vi "find_midle_lane_v3.vi"(8 "max_cluster_size":dbl=150.0 format="%#_13g", 9 "euclid":dbl=110.0, 10 "LiDAR_Y":i32[](array[numeric]), 11 "LiDAR_X":i32[](array[numeric])) -> (0 "크기":i32, 1 "lidar_x":dbl=-0.4638235294117647, 2 "ladpoint":cluster{dbl[], dbl[]}(graph)={[-463.8235294117647], [1690.0]}, 3 "filtered_data":cluster{dbl[], dbl[]}(graph)={[0.0, 0.0, 0.0, 0.0, 0.0, 0.0, 0.0, 0.0, 0.0, 0.0, 0.0, 0.0, 0.0, 0.0, 0.0, 0.0, 0.0, 200.0, 205.0, 210.0, 0.0, 0.0, 0.0, 0.0, 0.0, 0.0, 0.0, 0.0, 0.0, 0.0, 0.0, 0.0, 0.0, 0.0], [0.0, 0.0, 0.0, 0.0, 0.0, 0.0, 0.0, 0.0, 0.0, 0.0, 0.0, 0.0, 0.0, 0.0, 0.0, 0.0, 0.0, 500.0, 500.0, 500.0, 0.0, 0.0, 0.0, 0.0, 0.0, 0.0, 0.0, 0.0, 0.0, 0.0, 0.0, 0.0, 0.0, 0.0]}, 4 "right_point":dbl=-0.4638235294117647, 6 "left_point":dbl=-0.4638235294117647)   [LabVIEW 2024]
uses:
  <vilib>/Analysis/baseanly.llb/Mean (DBL).vi
  <vilib>/Analysis/NI_AALBase.lvlib
panel:
  out "raw_data":cluster{dbl[], dbl[]}(graph)
  out "배열":bool[](array[boolean])
  out "clustered_data1":cluster{dbl[], dbl[]}[](graph)=[{[0.0, 0.0, 0.0, 0.0, 0.0, 0.0, 0.0, 0.0, 0.0, 0.0, 0.0, 0.0, 0.0, 0.0, 0.0, 0.0, 0.0], [0.0, 0.0, 0.0, 0.0, 0.0, 0.0, 0.0, 0.0, 0.0, 0.0, 0.0, 0.0, 0.0, 0.0, 0.0, 0.0, 0.0]}, {[-600.0, -605.0, -400.0, -405.0, -200.0, -205.0, 0.0, 0.0, 0.0, 0.0, 0.0, 0.0, 0.0, 0.0, 0.0, 0.0, 0.0], [500.0, 500.0, 500.0, 500.0, 500.0, 500.0, 0.0, 0.0, 0.0, 0.0, 0.0, 0.0, 0.0, 0.0, 0.0, 0.0, 0.0]}, {[200.0, 205.0, 210.0, 0.0, 0.0, 0.0, 0.0, 0.0, 0.0, 0.0, 0.0, 0.0, 0.0, 0.0, 0.0, 0.0, 0.0], [500.0, 500.0, 500.0, 0.0, 0.0, 0.0, 0.0, 0.0, 0.0, 0.0, 0.0, 0.0, 0.0, 0.0, 0.0, 0.0, 0.0]}, {[500.0, 500.0, 500.0, 500.0, 500.0, 500.0, 500.0, 500.0, 500.0, 500.0, 500.0, 500.0, 500.0, 500.0, 500.0, 500.0, 500.0], [500.0, 700.0, 710.0, 720.0, 730.0, 740.0, 750.0, 760.0, 770.0, 780.0, 790.0, 800.0, 810.0, 820.0, 830.0, 840.0, 850.0]}, {[-250.0, -280.0, -290.0, -310.0, -330.0, -340.0, -360.0, -390.0, -410.0, -430.0, -440.0, 0.0, 0.0, 0.0, 0.0, 0.0, 0.0], [1100.0, 1100.0, 1100.0, 1100.0, 1100.0, 1100.0, 1100.0, 1100.0, 1100.0, 1100.0, 1100.0, 0.0, 0.0, 0.0, 0.0, 0.0, 0.0]}]
  out "clustered_data2":cluster{dbl[], dbl[]}(graph)={[0.0, 0.0, 0.0, 0.0, 0.0, 0.0, 0.0, 0.0, 0.0, 0.0, 0.0, 0.0, 0.0, 0.0, 0.0, 0.0, 0.0, 200.0, 205.0, 210.0, 0.0, 0.0, 0.0, 0.0, 0.0, 0.0, 0.0, 0.0, 0.0, 0.0, 0.0, 0.0, 0.0, 0.0], [0.0, 0.0, 0.0, 0.0, 0.0, 0.0, 0.0, 0.0, 0.0, 0.0, 0.0, 0.0, 0.0, 0.0, 0.0, 0.0, 0.0, 500.0, 500.0, 500.0, 0.0, 0.0, 0.0, 0.0, 0.0, 0.0, 0.0, 0.0, 0.0, 0.0, 0.0, 0.0, 0.0, 0.0]}
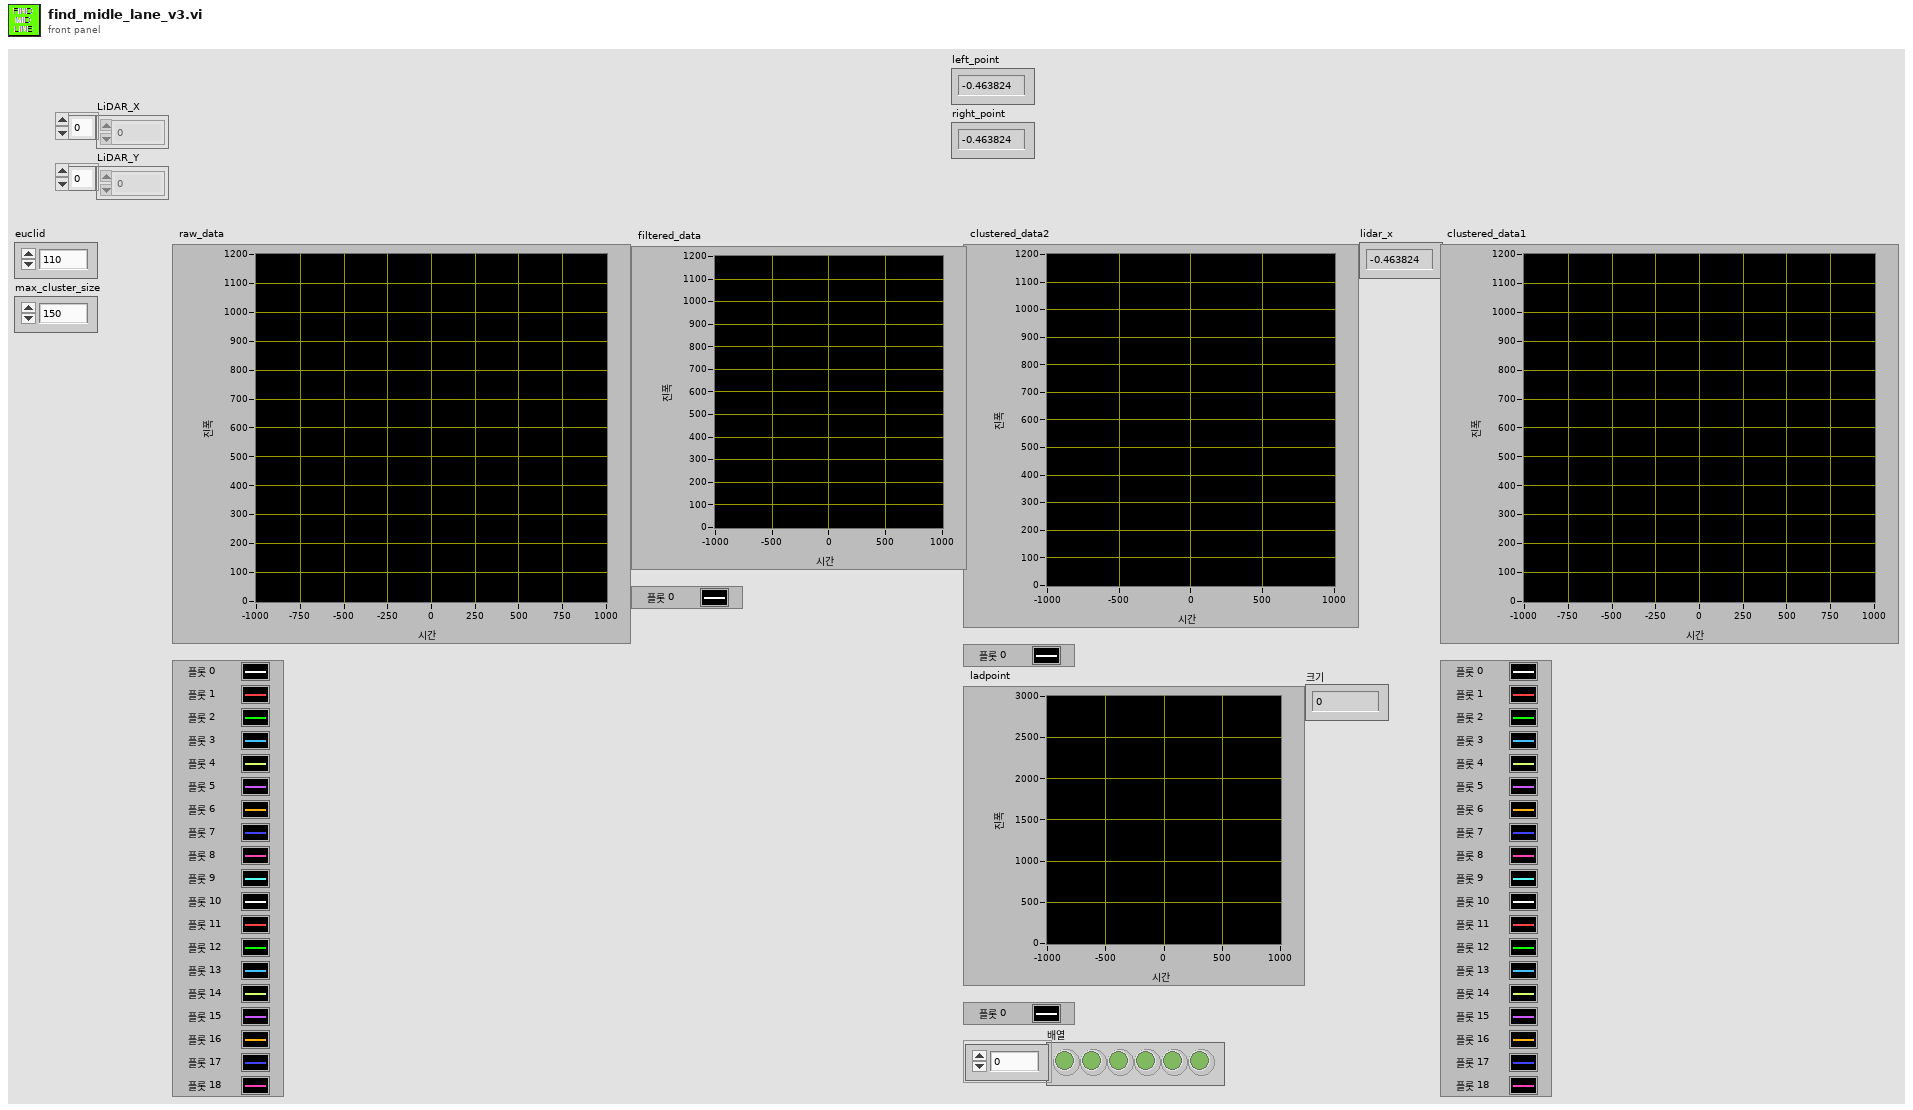
[diagram p1: front panel]
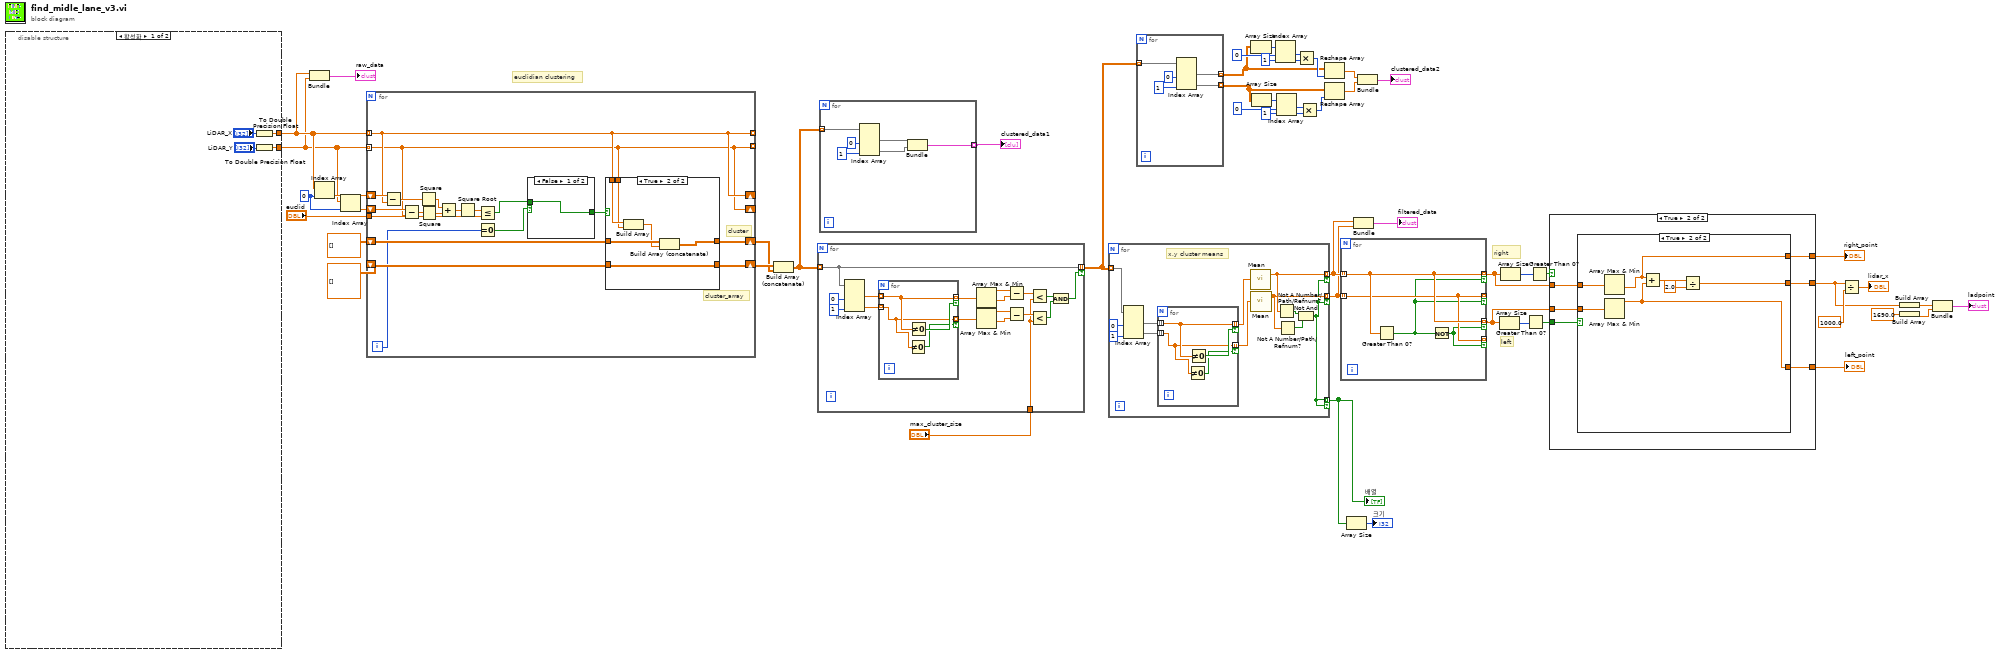
[diagram p0: block diagram]
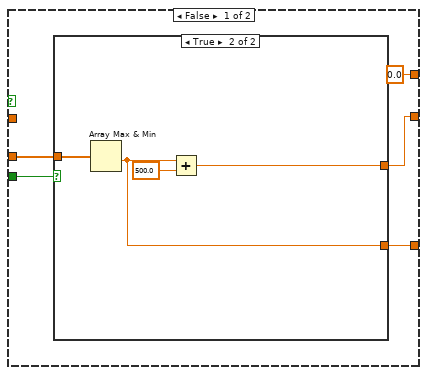
[diagram p2: hidden frame]
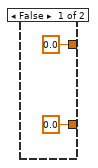
[diagram p3: hidden frame]
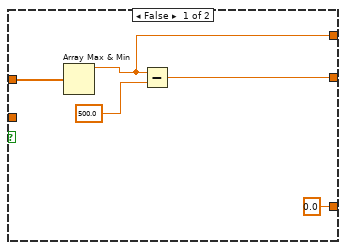
[diagram p4: hidden frame]
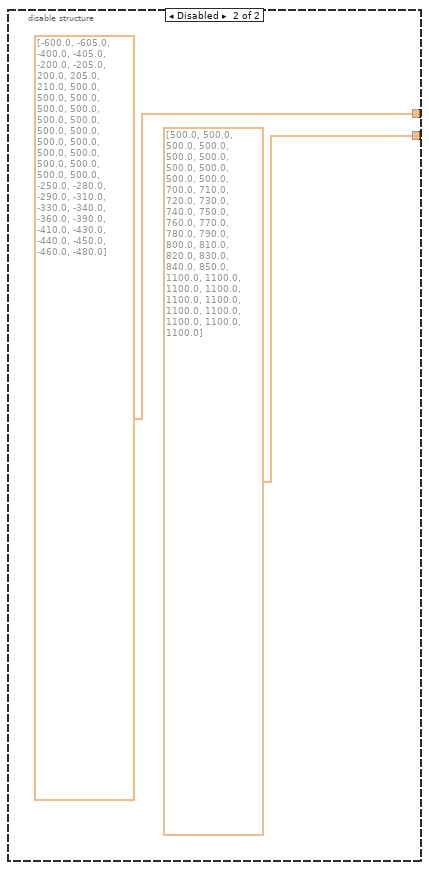
[diagram p5: hidden frame]
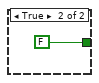
[diagram p6: hidden frame]
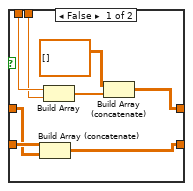
[diagram p7: hidden frame]
diagram:
  w47 = 0 ("인덱스")
  # "left"
  # "right"
  # "euclidian clustering"
  n1 = disable-structure shown="활성화" {
    disable-tunnel: [w54 dbl[] [500.0, 500.0, 500.0, 500.0, 500.0, 500.0, 500.0, 500.0, 500.0, 500.0, 700.0, 710.0, 720.0, 730.0, 740.0, 750.0, 760.0, 770.0, 780.0, 790.0, 800.0, 810.0, 820.0, 830.0, 840.0, 850.0, 1100.0, 1100.0, 1100.0, 1100.0, 1100.0, 1100.0, 1100.0, 1100.0, 1100.0, 1100.0, 1100.0]] -> w8
    disable-tunnel: [w53 dbl[] [-600.0, -605.0, -400.0, -405.0, -200.0, -205.0, 200.0, 205.0, 210.0, 500.0, 500.0, 500.0, 500.0, 500.0, 500.0, 500.0, 500.0, 500.0, 500.0, 500.0, 500.0, 500.0, 500.0, 500.0, 500.0, 500.0, -250.0, -280.0, -290.0, -310.0, -330.0, -340.0, -360.0, -390.0, -410.0, -430.0, -440.0, -450.0, -460.0, -480.0]] -> w9
    frame Enabled {
      n2 = To Double Precision Float(number="LiDAR_X") -> (double precision float=w53:dbl[])
      n3 = To Double Precision Float(number="LiDAR_Y") -> (double precision float=w54:dbl[])
    }
    frame Disabled {
    }
  }
  n4 = Bundle(w9, w8) -> (→"raw_data":cluster{dbl[], dbl[]})  [unwired: 1 in]
  n5 = Index Array(array=w9, index=w47) -> (element=w49:dbl)
  n6 = Index Array(array=w8, index=w47) -> (element=w48:dbl)
  n7 = for {
    tunnel: w9 -> [w66] mode=indexing
    tunnel: w8 -> [w65] mode=indexing
    tunnel: [w66] -> _ mode=indexing
    tunnel: [w65] -> _ mode=indexing
    shift-right: [w66] -> _
    shift-left: w49 -> [w77]
    shift-right: [w65] -> _
    shift-left: w48 -> [w76]
    tunnel: "euclid" -> [w69]
    shift-right: [w68] -> w30
    shift-left: dbl[][] [] -> [w67]
    shift-right: [w59] -> w31
    shift-left: dbl[][][] [] -> [w64]
    i -> [w63]
    # "cluster_array"
    # "cluster"
    n8 = Subtract(x=w77, y=w66) -> (x-y=w75:dbl)
    n9 = Subtract(x=w76, y=w65) -> (x-y=w74:dbl)
    n10 = Square(x=w75) -> (x^2=w73:dbl)
    n11 = Square(x=w74) -> (x^2=w72:dbl)
    n12 = Add(x=w73, y=w72) -> (x+y=w71:dbl)
    n13 = Square Root(x=w71) -> (sqrt(x)=w70:dbl)
    n14 = Equal To 0?(x=w63) -> (x = 0?=w62:bool)
    n15 = Less Or Equal?(x=w70, y=w69) -> (x <= y?=w60:bool)
    n16 = case shown="False" w62 {
      tunnel: [w78 FALSE] -> w61
      tunnel: w60 -> [w78 _]
      frame False {
      }
      frame True {
      }
    }
    n17 = case shown="True" w61 {
      tunnel: [w83 w93] -> w68
      tunnel: w67 -> [w81 w92]
      tunnel: [w80 w88] -> w59
      tunnel: w66 -> [w86 w91]
      tunnel: w65 -> [w85 w90]
      tunnel: w64 -> [w82 w88]
      frame False {
        n18 = Build Array (concatenate)(w82, w81) -> (w80:dbl[][][])
        n19 = Build Array(w86, w85) -> (w84:dbl[])
        n20 = Build Array (concatenate)(dbl[][] [], w84) -> (w83:dbl[][])
      }
      frame True {
        n21 = Build Array(w91, w90) -> (w89:dbl[])
        n22 = Build Array (concatenate)(w92, w89) -> (w93:dbl[][])
      }
    }
  }
  n23 = Build Array (concatenate)(w31, w30) -> (w16:dbl[][][])
  n24 = for {
    tunnel: w16 -> [w106] mode=indexing
    tunnel: [w106] -> w6 mode=indexing if=w101
    tunnel: "max_cluster_size" -> [w94]
    n25 = Index Array(array=w106, index (col) #1=0 ("비활성화된 인덱스 (열)"), index (col) #2=1 ("인덱스 (열)")) -> (element #1=w98:dbl[], element #2=w97:dbl[])  [unwired: 2 in]
    n26 = for {
      tunnel: w98 -> [w114] mode=indexing
      tunnel: w97 -> [w112] mode=indexing
      tunnel: [w114] -> w96 mode=indexing if=w113
      tunnel: [w112] -> w95 mode=indexing if=w111
      n27 = Not Equal To 0?(x=w112) -> (x != 0?=w111:bool)
      n28 = Not Equal To 0?(x=w114) -> (x != 0?=w113:bool)
    }
    n29 = Array Max & Min(array=w95) -> (max value=w103:dbl, min value=w102:dbl)  [unwired: 2 out]
    n30 = Array Max & Min(array=w96) -> (max value=w105:dbl, min value=w104:dbl)  [unwired: 2 out]
    n31 = Subtract(x=w105, y=w104) -> (x-y=w100:dbl)
    n32 = Subtract(x=w103, y=w102) -> (x-y=w99:dbl)
    n33 = Less?(x=w100, y=w94) -> (x < y?=w108:bool)
    n34 = Less?(x=w99, y=w94) -> (x < y?=w107:bool)
    n35 = And(x=w108, y=w107) -> (x .and. y?=w101:bool)
  }
  n36 = for {
    tunnel: w16 -> [w120] mode=indexing
    tunnel: [w115] -> w17 mode=indexing
    n37 = Index Array(array=w120, index (col) #1=0 ("인덱스"), index (col) #2=1 ("인덱스")) -> (element #1=w117:dbl[], element #2=w116:dbl[])  [unwired: 2 in]
    n38 = Bundle(w117, w116) -> (w115:cluster{dbl[], dbl[]})  [unwired: 1 in]
  }
  "clustered_data1" <- w17
  n39 = for {
    tunnel: w6 -> [w128] mode=indexing
    tunnel: [w125] -> w14 mode=indexing if=w121
    tunnel: [w124] -> w13 mode=indexing if=w121
    tunnel: [w121] -> w11 mode=indexing if=w121
    # "x,y cluster means"
    n40 = Index Array(array=w128, index (col) #1=0 ("비활성화된 인덱스 (열)"), index (col) #2=1 ("인덱스 (열)")) -> (element #1=w131:dbl[], element #2=w132:dbl[])  [unwired: 2 in]
    n41 = for {
      tunnel: w131 -> [w136] mode=indexing
      tunnel: w132 -> [w134] mode=indexing
      tunnel: [w136] -> w127 mode=indexing if=w135
      tunnel: [w134] -> w126 mode=indexing if=w133
      n42 = Not Equal To 0?(x=w134) -> (x != 0?=w133:bool)
      n43 = Not Equal To 0?(x=w136) -> (x != 0?=w135:bool)
    }
    n44 = call-poly <vilib>:"Mean.vi"("X"=w127) -> ("mean"=w125:dbl)  [unwired: 1 out]
    n45 = call-poly <vilib>:"Mean.vi"("X"=w126) -> ("mean"=w124:dbl)  [unwired: 1 out]
    n46 = Not A Number/Path/Refnum?(number/path/refnum=w125) -> (NaN/Path/Refnum?=w123:bool)
    n47 = Not A Number/Path/Refnum?(number/path/refnum=w124) -> (NaN/Path/Refnum?=w122:bool)
    n48 = Not And(1:w122, 2:w123) -> (0:w121:bool)
  }
  "배열" <- w11
  n49 = for {
    tunnel: w6 -> [w141] mode=indexing
    tunnel: [w138] -> w19 mode=indexing
    tunnel: [w137] -> w18 mode=indexing
    n50 = Index Array(array=w141, index (col) #1=0 ("인덱스"), index (col) #2=1 ("인덱스")) -> (element #1=w138:dbl[], element #2=w137:dbl[])  [unwired: 2 in]
  }
  n51 = Array Size(array=w19) -> (size(s)=w44:i32[])
  n52 = Array Size(array=w18) -> (size(s)=w39:i32[])
  n53 = Index Array(array=w44, index #1=0 ("인덱스"), index #2=1 ("인덱스")) -> (element #1=w34:i32, element #2=w35:i32)
  n54 = Index Array(array=w39, index #1=0 ("인덱스"), index #2=1 ("인덱스")) -> (element #1=w38:i32, element #2=w37:i32)
  n55 = Multiply(x=w34, y=w35) -> (x*y=w33:i32)
  n56 = Multiply(x=w38, y=w37) -> (x*y=w36:i32)
  n57 = Reshape Array(w19, w33) -> (w46:dbl[])
  n58 = Reshape Array(w18, w36) -> (w45:dbl[])
  n59 = for {
    tunnel: w14 -> [w145] mode=indexing
    tunnel: w13 -> [w144] mode=indexing
    tunnel: [w145] -> w5 mode=indexing if=w143
    tunnel: [w144] -> _ mode=indexing if=w143
    tunnel: [w145] -> w4 mode=indexing if=w142
    tunnel: [w144] -> _ mode=indexing if=w142
    n60 = Greater Than 0?(x=w145) -> (x > 0?=w143:bool)
    n61 = Not(x=w143) -> (.not. x?=w142:bool)
  }
  n62 = Array Size(array=w11) -> (size(s)=→"크기":i32)
  n63 = Bundle(w14, w13) -> (→"filtered_data":cluster{dbl[], dbl[]})  [unwired: 1 in]
  n64 = Bundle(w46, w45) -> (→"clustered_data2":cluster{dbl[], dbl[]})  [unwired: 1 in]
  n65 = Array Size(array=w4) -> (size(s)=w28:i32)
  n66 = Array Size(array=w5) -> (size(s)=w29:i32)
  n67 = Greater Than 0?(x=w28) -> (x > 0?=w26:bool)
  n68 = Greater Than 0?(x=w29) -> (x > 0?=w27:bool)
  n69 = case shown="True" w27 {
    tunnel: w26 -> [w150 w162]
    tunnel: w4 -> [w149 w161]
    tunnel: w5 -> [_ w160]
    tunnel: [w148 w159] -> w20
    tunnel: [0.0 w158] -> w2
    tunnel: [w146 w157] -> w1
    frame False {
      n70 = case shown="True" w150 {
        tunnel: w149 -> [_ w156]
        tunnel: [0.0 w154] -> w148
        tunnel: [0.0 w153] -> w146
        frame False {
        }
        frame True {
          n71 = Array Max & Min(array=w156) -> (min value=w153:dbl)  [unwired: 3 out]
          n72 = Add(x=w153, y=500.0) -> (x+y=w154:dbl)
        }
      }
    }
    frame True {
      n73 = case shown="True" w162 {
        tunnel: w161 -> [_ w174]
        tunnel: w160 -> [w167 w173]
        tunnel: [w165 w170] -> w159
        tunnel: [w164 w169] -> w158
        tunnel: [0.0 w168] -> w157
        frame False {
          n74 = Array Max & Min(array=w167) -> (max value=w164:dbl)  [unwired: 3 out]
          n75 = Subtract(x=w164, y=500.0) -> (x-y=w165:dbl)
        }
        frame True {
          n76 = Array Max & Min(array=w173) -> (min value=w169:dbl)  [unwired: 3 out]
          n77 = Array Max & Min(array=w174) -> (max value=w168:dbl)  [unwired: 3 out]
          n78 = Add(x=w169, y=w168) -> (x+y=w172:dbl)
          n79 = Divide(x=w172, y=2.0) -> (x/y=w170:dbl)
        }
      }
    }
  }
  "left_point" <- w1
  "right_point" <- w2
  n80 = Divide(x=w20, y=1000.0) -> (x/y=→"lidar_x":dbl)
  n81 = Build Array(w20) -> (w22:dbl[])
  n82 = Build Array(1690.0 ("원소")) -> (w21:dbl[])
  n83 = Bundle(w22, w21) -> (→"ladpoint":cluster{dbl[], dbl[]})  [unwired: 1 in]
